vi "Window_Move.vi"(0 "VI":refnum<vi>, 5 "DX":i32, 7 "DY":i32, 11 "error in":errorcluster) -> (15 "error out":errorcluster)   [LabVIEW 2020, in "GH_App.lvlib"]
doc: "Moves the window of the VI by DX, DY pixels (Front Panel Window:Panel Bounds) - for dragging Main by its top border."
uses:
  GH_App.lvlib
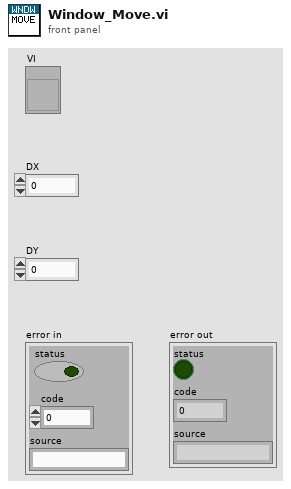
[diagram p1: front panel]
types:
  T1 = typedef "LVRectTypeDef.ctl" = cluster{"left":i16, "top":i16, "right":i16, "bottom":i16}
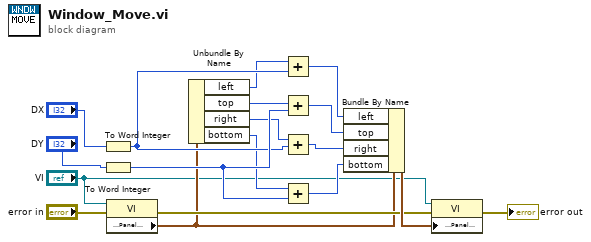
[diagram p0: block diagram]
diagram:
  n1 = To Word Integer(number="DX") -> (16bit integer=w11:i16)
  n2 = To Word Integer(number="DY") -> (16bit integer=w12:i16)
  n3 = property class="VI"(reference="VI", error in="error in") -> (error out=w6:errorcluster, "Front Panel Window:Panel Bounds"=w5:T1)  [unwired: 1 out]
  n4 = Unbundle By Name(w5) -> ("left"=w7:i16, "top"=w8:i16, "right"=w9:i16, "bottom"=w10:i16)
  n5 = Add(x=w7, y=w11) -> (x+y=w13:i16)
  n6 = Add(x=w8, y=w12) -> (x+y=w14:i16)
  n7 = Add(x=w9, y=w11) -> (x+y=w15:i16)
  n8 = Add(x=w10, y=w12) -> (x+y=w16:i16)
  n9 = Bundle By Name(cluster=w5, "left"=w13, "top"=w14, "right"=w15, "bottom"=w16) -> (w17:T1)
  n10 = property class="VI"(reference="VI", error in=w6, "Front Panel Window:Panel Bounds"=w17) -> (error out=→"error out":errorcluster)  [unwired: 1 out]
